vi "Trimming_Coil_Ramps.vi"() -> ()   [LabVIEW 2025]
panel:
  out "Cluster":T1
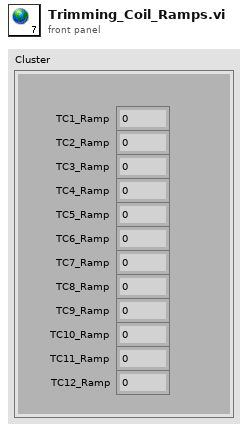
[diagram p1: front panel]
types:
  T1 = cluster{"TC1_Ramp":dbl, "TC2_Ramp":dbl, "TC3_Ramp":dbl, "TC4_Ramp":dbl, "TC5_Ramp":dbl, "TC6_Ramp":dbl, "TC7_Ramp":dbl, "TC8_Ramp":dbl, "TC9_Ramp":dbl, "TC10_Ramp":dbl, "TC11_Ramp":dbl, "TC12_Ramp":dbl}
diagram:
